vi "VIH XML - Enum Values to-from XML String.vi"(6 "cmd (check)":enum16{"check", "parse", "format"}(ring), 8 "error in":errorcluster, 10 "Enum Values in":T1[](array[typedef]), 11 "XML in":string) -> (0 "error out":errorcluster, 1 "available":bool, 2 "Enum Values out":T1[](array[typedef]), 3 "XML out":string)   [LabVIEW 2014]
doc: "::: VI Helpeks :::\nCopyright (c) 2000-2026 Konstantin Shifershteyn. All rights reserved."
uses:
  _VIH HelpGen.llb/VIH HelpGen Typedef - Cluster - Enum Value Info.ctl
  <vilib>/xml/Close Reference(Node).vi
  <vilib>/xml/NI_XML.lvlib
  <resource>/objmgr/DOMUserDefRef.rc
panel:
  # "VI Helpeks\nCopyright (c) 2012-2026 Konstantin Shifershteyn"
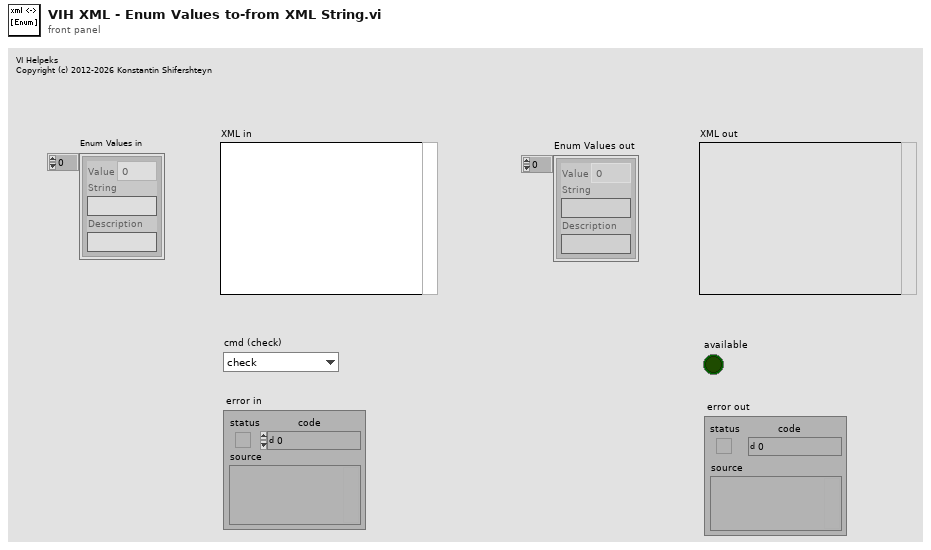
[diagram p1: front panel]
types:
  T1 = typedef "VIH HelpGen Typedef - Cluster - Enum Value Info.ctl" = cluster{"Value":ext, "String":string, "Description":string}
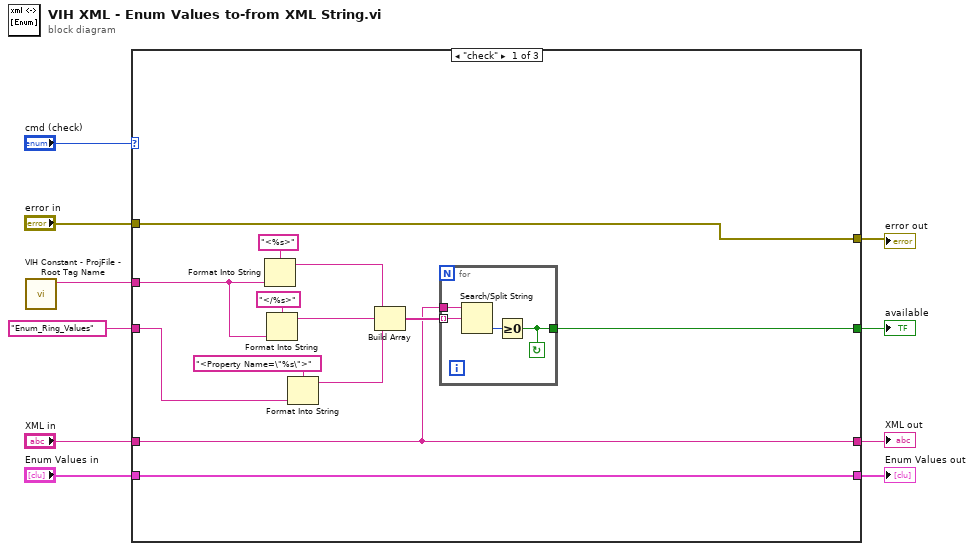
[diagram p0: block diagram]
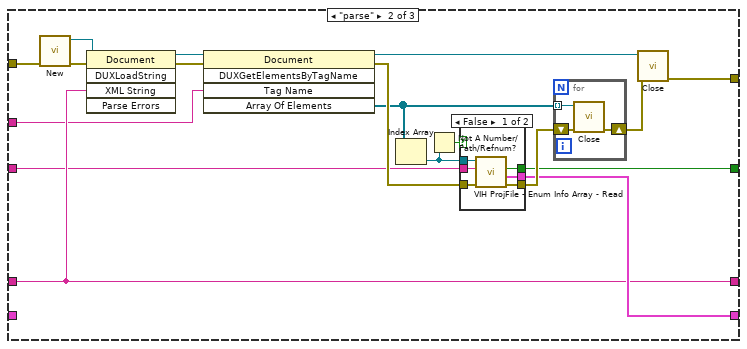
[diagram p2: hidden frame]
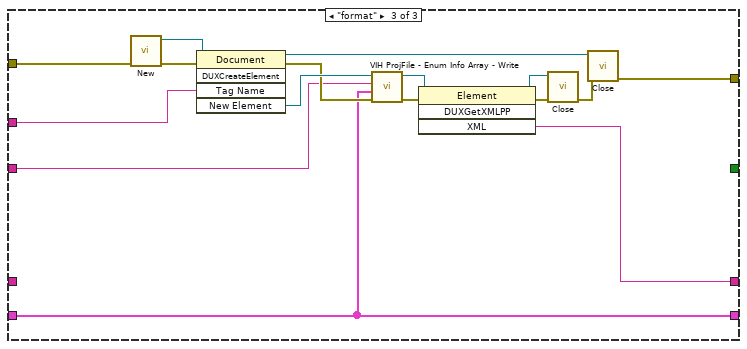
[diagram p4: hidden frame]
diagram:
  n1 = call "VIH Constant - ProjFile - Root Tag Name.vi"() -> ("Tag Name"=w1:string)  [unwired: 11 in]
  n2 = case shown="\"check\"" "cmd (check)" {
    tunnel: "error in" -> [w23 w34 w61]
    tunnel: "Enum Values in" -> [w22 _ w56]
    tunnel: [w23 w33 w60] -> w7
    tunnel: [w17 w31 w59] -> w6
    tunnel: [w22 w32 w56] -> w5
    tunnel: "XML in" -> [w17 w31 _]
    tunnel: w1 -> [w13 w30 w58]
    tunnel: "Enum_Ring_Values" ("Property Name") -> [w11 w29 w57]
    tunnel: [w18 w28 _] -> w2
    frame "check" {
      n3 = Format Into String(format string="<%s>", w13) -> (resulting string=w16:string)  [unwired: 2 in, 1 out]
      n4 = Format Into String(format string="</%s>", w13) -> (resulting string=w15:string)  [unwired: 2 in, 1 out]
      n5 = Format Into String(format string="<Property Name=\"%s\">", w11) -> (resulting string=w12:string)  [unwired: 2 in, 1 out]
      n6 = Build Array(w16, w15, w12) -> (w21:string[])
      n7 = for {
        tunnel: w21 -> [w25] mode=indexing
        tunnel: [w26] -> w18
        tunnel: w17 -> [w24]
        stop <- w26 continue-if-true
        n8 = Search/Split String(string=w24, search string/char (-)=w25) -> (offset of match=w27:i32)  [unwired: 1 in, 2 out]
        n9 = Greater Or Equal To 0?(x=w27) -> (x >= 0?=w26:bool)
      }
    }
    frame "parse" {
      n10 = call <vilib>:"New.vi"("error in (no error)"=w34) -> ("error out"=w44:errorcluster, "DOM document out"=w45:refnum<k20>)  [unwired: 7 in]
      n11 = invoke class="Document" method="DUXLoadString"(reference=w45, error in=w44, "XML String"=w31) -> (reference out=w42:refnum<k20>, error out=w41:errorcluster)  [unwired: 2 in, 3 out]
      n12 = invoke class="Document" method="DUXGetElementsByTagName"(reference=w42, error in=w41, "Tag Name"=w30) -> (reference out=w39:refnum<k20>, error out=w40:errorcluster, "Array Of Elements"=w38:refnum<k20>[])  [unwired: 2 in, 2 out]
      n13 = Index Array(array=w38) -> (element=w36:refnum<k20>)  [unwired: 1 in]
      n14 = Not A Number/Path/Refnum?(number/path/refnum=w36) -> (NaN/Path/Refnum?=w35:bool)
      n15 = case shown="False" w35 {
        tunnel: w29 -> [w51 _]
        tunnel: [w50 _] -> w32
        tunnel: w40 -> [w49 w52]
        tunnel: [w48 w52] -> w37
        tunnel: w36 -> [w47 _]
        tunnel: [w46 _] -> w28
        frame False {
          n16 = call "VIH ProjFile - Enum Info Array - Read.vi"("error in"=w49, "Property Name"=w51, "XML Parent Item"=w47) -> ("error out"=w48:errorcluster, "EnumValDscr"=w50:T1[], "Property found"=w46:bool)  [unwired: 5 in, 1 out]
        }
        frame True {
        }
      }
      n17 = for {
        tunnel: w38 -> [w54] mode=indexing
        shift-right: [w55] -> w43
        shift-left: w37 -> [w53]
        n18 = call-poly <vilib>:"Close.vi"("error in (no error)"=w53, "node"=w54) -> ("error out"=w55:errorcluster)  [unwired: 7 in]
      }
      n19 = call-poly <vilib>:"Close.vi"("error in (no error)"=w43, "node"=w39) -> ("error out"=w33:errorcluster)  [unwired: 7 in]
    }
    frame "format" {
      n20 = call <vilib>:"New.vi"("error in (no error)"=w61) -> ("error out"=w67:errorcluster, "DOM document out"=w70:refnum<k20>)  [unwired: 7 in]
      n21 = invoke class="Document" method="DUXCreateElement"(reference=w70, error in=w67, "Tag Name"=w58) -> (reference out=w68:refnum<k20>, error out=w69:errorcluster, "New Element"=w71:refnum<k20>)  [unwired: 2 in, 2 out]
      n22 = call "VIH ProjFile - Enum Info Array - Write.vi"("error in"=w69, "EnumValDscr"=w56, "Property Name"=w57, "XML Parent Item"=w71) -> ("error out"=w63:errorcluster, "dup XML Parent Item"=w62:refnum<k20>)  [unwired: 6 in]
      n23 = invoke class="Element" method="DUXGetXMLPP"(reference=w62, error in=w63) -> (reference out=w65:refnum<k20>, error out=w64:errorcluster, "XML"=w59:string)  [unwired: 2 in, 1 out]
      n24 = call-poly <vilib>:"Close.vi"("error in (no error)"=w64, "node"=w65) -> ("error out"=w66:errorcluster)  [unwired: 7 in]
      n25 = call-poly <vilib>:"Close.vi"("error in (no error)"=w66, "node"=w68) -> ("error out"=w60:errorcluster)  [unwired: 7 in]
    }
  }
  "Enum Values out" <- w5
  "XML out" <- w6
  "error out" <- w7
  "available" <- w2
